vi "BNAL RADAR graph Formation.vi"(8 "Cutted Sample Sequence":string="TCTAGACTATCTCACTCTCAGATGAGATCGATAGATCAGT", 9 "Level Composition":string[](array[string]), 11 "Assigned#_CL":T1) -> (0 "Base_Tag_Array":string[](array[string]), 1 "Base_Com_Array":i32[](array[numeric]), 2 "Table Cluster":T2, 3 "Radar graph cluster":T3)   [LabVIEW 2018]
uses:
  a6b6b03c-adef-4b05-a669-847ce0550db9.vi
  4a9d2bae-dd06-40cf-8326-d887beb1304b.vi
  f1d95cbe-b5e7-4193-9626-4301581f2f47.vi
  <vilib>/Array/Sort 2D Array - Pop Stack.vi
  <vilib>/Array/Sort 2D Array - Push Stack.vi
panel:
  out "Tri_N_sort_#":string[](array[string])
  out "Tri_P_sort_#":string[](array[string])
  out "Di_N_sort_#":string[](array[string])
  out "Di_P_sort_#":string[](array[string])
  out "Mono_N_sort_#":string[](array[string])
  out "Mono_P_sort_#":string[](array[string])
  out "Tri Table":string[][](table)
  out "Di Table":string[][](table)
  out "Mono Table":string[][](table)
  out "Mono_N_sort_B":string[](array[string])
  out "Mono_P_sort_B":string[](array[string])
  out "Mono_P_sort_[%]":string[](array[string])
  out "Mono_N_sort_[%]":string[](array[string])
  out "Tri_N_sort_B":string[](array[string])
  out "Tri_P_sort_B":string[](array[string])
  out "Tri_P_sort_[%]":string[](array[string])
  out "Tri_N_sort_[%]":string[](array[string])
  out "Di_N_sort_B":string[](array[string])
  out "Di_P_sort_B":string[](array[string])
  out "Di_P_sort_[%]":string[](array[string])
  out "Di_N_sort_[%]":string[](array[string])
  out "Tri_sort_B":string[](array[string])
  out "Tri_sort":dbl[](array[numeric])
  out "Tri_Assig-Th":dbl[](array[numeric])
  out "TriBase_Array_Tag":string[](array[string])
  out "Di_sort_B":string[](array[string])
  out "Di_sort":dbl[](array[numeric])
  out "Mono_sort_B":string[](array[string])
  out "Mono_sort":dbl[](array[numeric])
  out "DiBase_Array_Tag":string[](array[string])
  out "MonoBase_Array_Tag":string[](array[string])
  out "Di_MxR-Th":dbl[](array[numeric])
  out "Mono_MxR-Th":dbl[](array[numeric])
  out "Di_Assig-Th":dbl[](array[numeric])
  out "Mono_Assig-Th":dbl[](array[numeric])
  out "Tri_Theory[%]":dbl[](array[numeric])
  out "Di_Theory[%]":dbl[](array[numeric])
  out "Mono_Theory[%]":dbl[](array[numeric])
  out "Tri_MxRight[%]":dbl[](array[numeric])
  out "Di_MxRight[%]":dbl[](array[numeric])
  out "Mono_MxRight[%]":dbl[](array[numeric])
  out "Tri_Assigned[%]":dbl[](array[numeric])
  out "Di_Assigned[%]":dbl[](array[numeric])
  out "Mono_Assigned[%]":dbl[](array[numeric])
  out "Tri_MxRight#":i32[](array[numeric])
  out "Di_MxRight#":i32[](array[numeric])
  out "Mono_MxRight#":i32[](array[numeric])
  out "Tri_Assigned#":i32[](array[numeric])
  out "Di_Assigned#":i32[](array[numeric])
  out "Mono_Assigned#":i32[](array[numeric])
  out "Radar Plot_XXX":picture
  out "Radar Plot_XX":picture
  out "Radar_X":picture
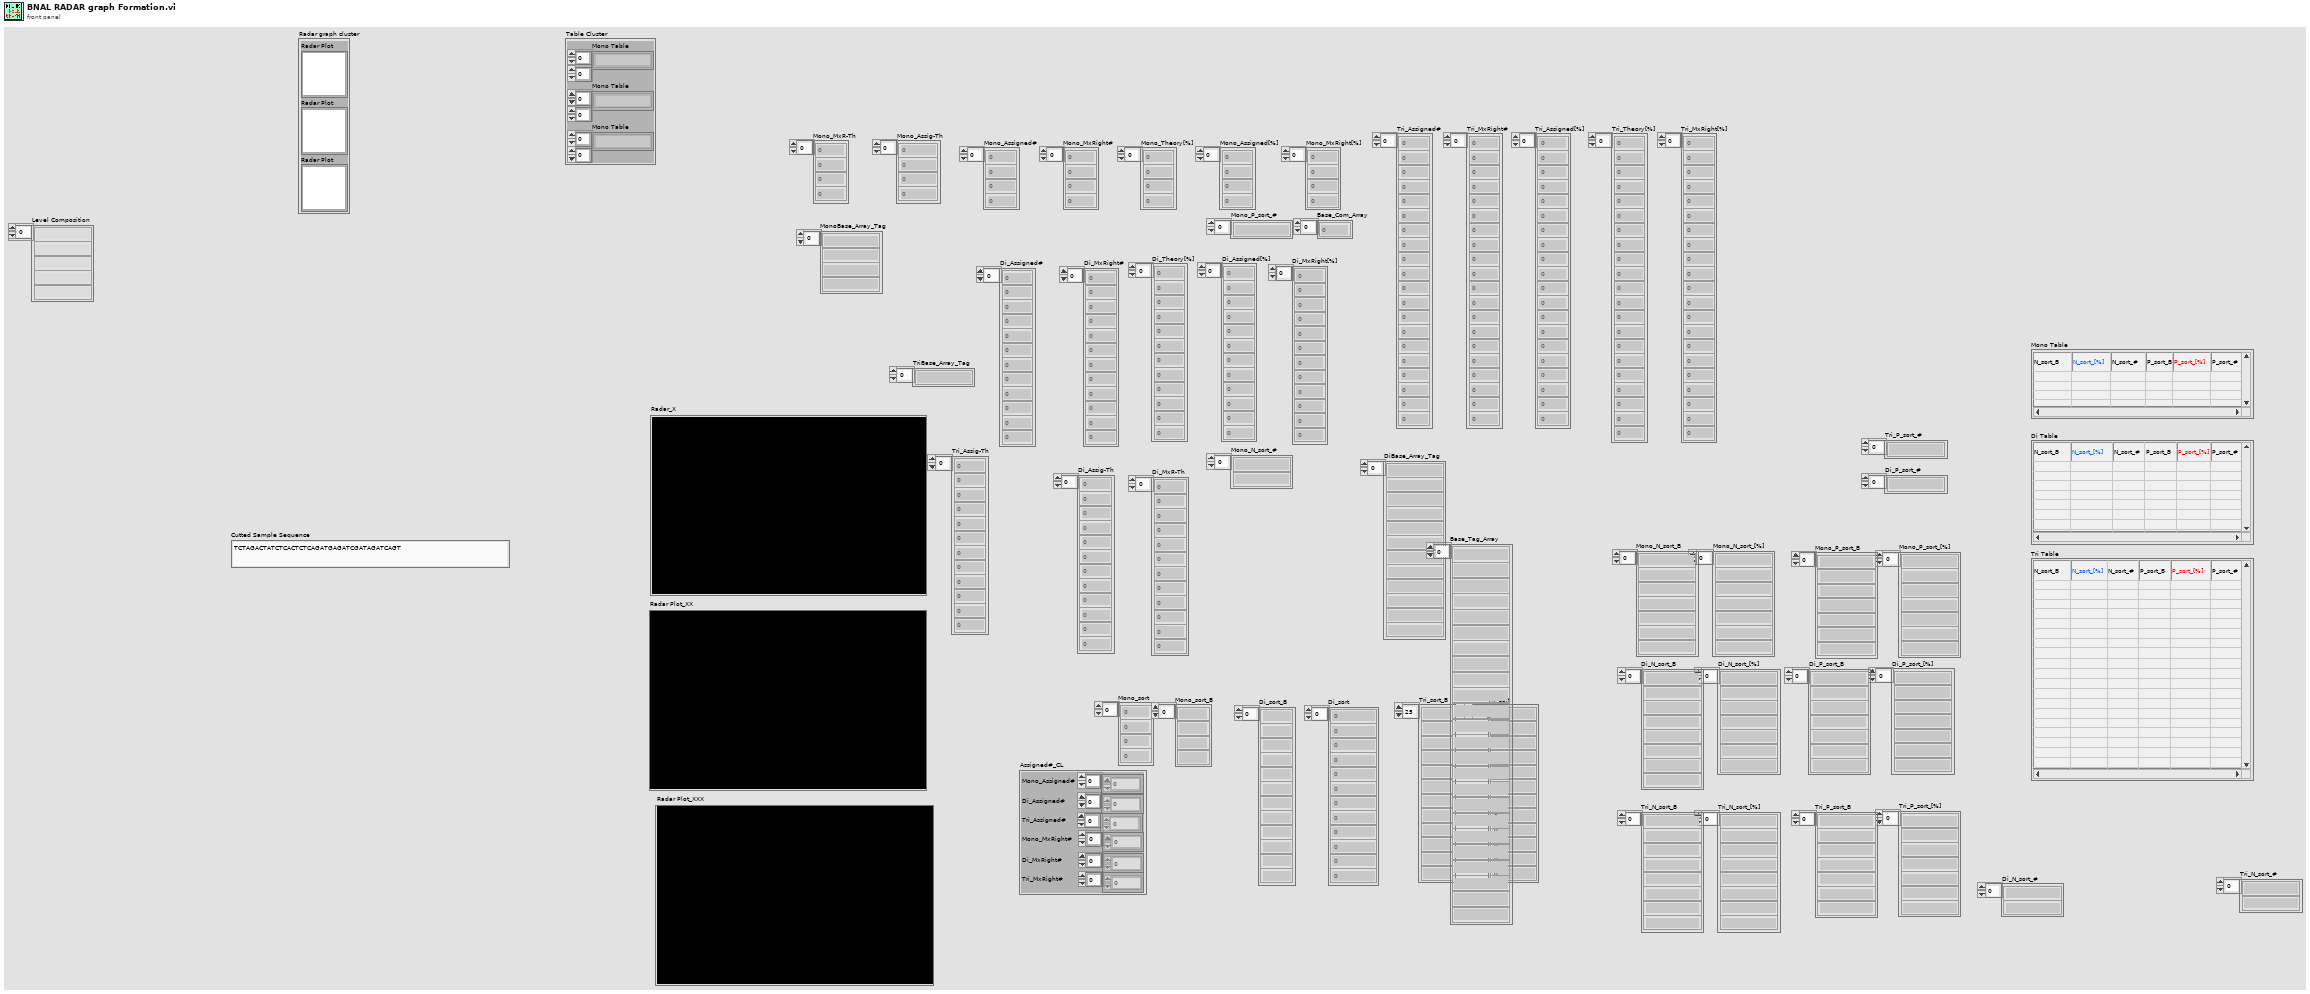
[diagram p1: front panel]
types:
  T1 = cluster{"Mono_Assigned#":i32[], "Di_Assigned#":i32[], "Tri_Assigned#":i32[], "Tri_MxRight#":i32[], "Di_MxRight#":i32[], "Mono_MxRight#":i32[]}
  T2 = cluster{"Mono Table":string[][], "Mono Table":string[][], "Mono Table":string[][]}
  T3 = cluster{"Radar Plot":picture, "Radar Plot":picture, "Radar Plot":picture}
  T4 = cluster{"MonoBase_Array_Tag":string[], "DiBase_Array_Tag":string[], "TriBase_Array_Tag":string[]}
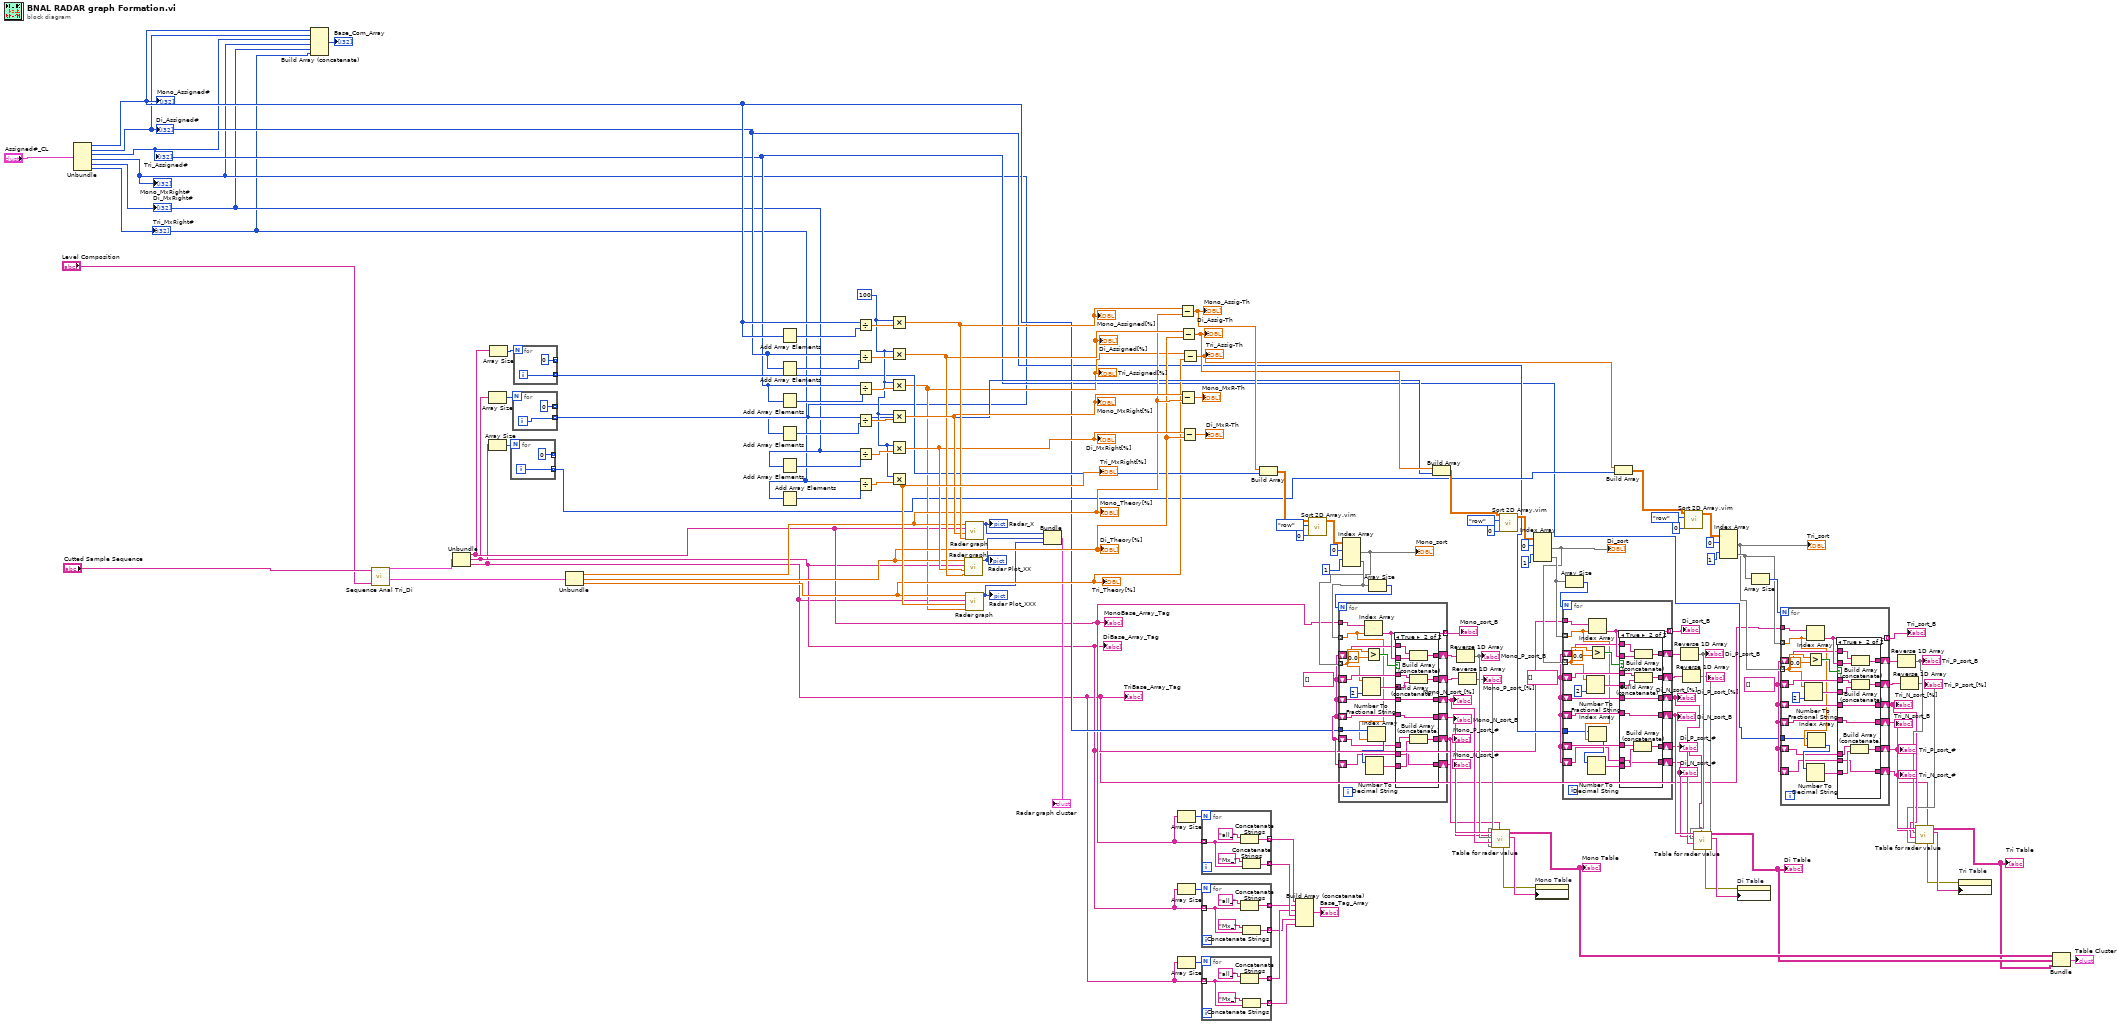
[diagram p0: block diagram]
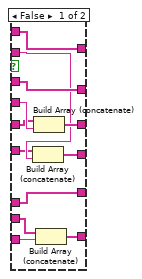
[diagram p2: hidden frame]
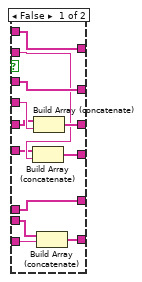
[diagram p3: hidden frame]
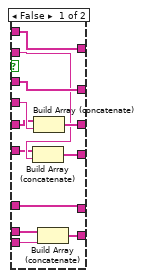
[diagram p4: hidden frame]
diagram:
  w38 = string[] []
  w36 = string[] []
  w37 = string[] []
  w110 = 100
  n1 = Unbundle("Assigned#_CL") -> ("Mono_Assigned#"=w20:i32[], "Di_Assigned#"=w19:i32[], "Tri_Assigned#"=w18:i32[], "Tri_MxRight#"=w17:i32[], "Di_MxRight#"=w16:i32[], "Mono_MxRight#"=w15:i32[])
  "Mono_Assigned#" <- w20
  "Di_Assigned#" <- w19
  "Tri_Assigned#" <- w18
  "Mono_MxRight#" <- w17
  "Di_MxRight#" <- w16
  "Tri_MxRight#" <- w15
  n2 = Build Array (concatenate)(w20, w19, w18, w17, w16, w15) -> (→"Base_Com_Array":i32[])
  n3 = call "Sequence Anal Tri_Di.vi"("Level Composition"="Level Composition", "String"="Cutted Sample Sequence") -> ("B%Number"=w127:cluster{dbl[], dbl[], dbl[]}, "Base Tag"=w128:T4)  [unwired: 7 in, 1 out]
  n4 = Unbundle(w128) -> ("MonoBase_Array_Tag"=w3:string[], "DiBase_Array_Tag"=w2:string[], "TriBase_Array_Tag"=w1:string[])
  "MonoBase_Array_Tag" <- w3
  "DiBase_Array_Tag" <- w2
  "TriBase_Array_Tag" <- w1
  n5 = Array Size(array=w2) -> (size(s)=w118:i32)
  n6 = Array Size(array=w1) -> (size(s)=w117:i32)
  n7 = Array Size(array=w3) -> (size(s)=w119:i32)
  n8 = for {
    N: w117 -> [_]
    tunnel: [0 ("index")] -> _ mode=indexing
    tunnel: [w130] -> w73 mode=indexing
    i -> [w130]
  }
  n9 = for {
    N: w118 -> [_]
    tunnel: [0 ("index")] -> _ mode=indexing
    tunnel: [w132] -> w91 mode=indexing
    i -> [w132]
  }
  n10 = for {
    N: w119 -> [_]
    tunnel: [0 ("index")] -> _ mode=indexing
    tunnel: [w134] -> w99 mode=indexing
    i -> [w134]
  }
  n11 = Unbundle(w127) -> (w102:dbl[], w101:dbl[], w81:dbl[])
  "Mono_Theory[%]" <- w102
  "Di_Theory[%]" <- w101
  "Tri_Theory[%]" <- w81
  n12 = Add Array Elements(numeric array=w20) -> (sum=w126:i32)
  n13 = Add Array Elements(numeric array=w19) -> (sum=w124:i32)
  n14 = Add Array Elements(numeric array=w18) -> (sum=w123:i32)
  n15 = Add Array Elements(numeric array=w17) -> (sum=w116:i32)
  n16 = Add Array Elements(numeric array=w16) -> (sum=w114:i32)
  n17 = Add Array Elements(numeric array=w15) -> (sum=w113:i32)
  n18 = Divide(x=w20, y=w126) -> (x/y=w125:dbl[])
  n19 = Divide(x=w19, y=w124) -> (x/y=w122:dbl[])
  n20 = Divide(x=w18, y=w123) -> (x/y=w121:dbl[])
  n21 = Divide(x=w17, y=w116) -> (x/y=w115:dbl[])
  n22 = Divide(x=w16, y=w114) -> (x/y=w112:dbl[])
  n23 = Divide(x=w15, y=w113) -> (x/y=w111:dbl[])
  n24 = Multiply(x=w110, y=w125) -> (x*y=w108:dbl[])
  "Mono_Assigned[%]" <- w108
  n25 = Multiply(x=w110, y=w122) -> (x*y=w106:dbl[])
  "Di_Assigned[%]" <- w106
  n26 = Multiply(x=w110, y=w121) -> (x*y=w80:dbl[])
  "Tri_Assigned[%]" <- w80
  n27 = Multiply(x=w110, y=w115) -> (x*y=w107:dbl[])
  "Mono_MxRight[%]" <- w107
  n28 = Multiply(x=w110, y=w112) -> (x*y=w104:dbl[])
  "Di_MxRight[%]" <- w104
  n29 = Multiply(x=w110, y=w111) -> (x*y=w109:dbl[])
  "Tri_MxRight[%]" <- w109
  n30 = call "Rader graph.vi"("Real B_Comp (NR)"=w106, "Real B_Comp (RR)"=w104, "XBase_Array_Tag"=w2, "Theory B_Comp"=w101) -> ("Radar Plot"=w28:picture)  [unwired: 7 in]
  "Radar Plot_XX" <- w28
  n31 = call "Rader graph.vi"("Real B_Comp (NR)"=w108, "Real B_Comp (RR)"=w107, "XBase_Array_Tag"=w3, "Theory B_Comp"=w102) -> ("Radar Plot"=w29:picture)  [unwired: 7 in]
  "Radar_X" <- w29
  n32 = call "Rader graph.vi"("Real B_Comp (NR)"=w80, "Real B_Comp (RR)"=w109, "XBase_Array_Tag"=w1, "Theory B_Comp"=w81) -> ("Radar Plot"=w27:picture)  [unwired: 7 in]
  "Radar Plot_XXX" <- w27
  n33 = Bundle("Radar Plot"=w29, "Radar Plot"=w28, "Radar Plot"=w27) -> (→"Radar graph cluster":T3)  [unwired: 1 in]
  n34 = Array Size(array=w3) -> (size(s)=w13:i32)
  n35 = Array Size(array=w2) -> (size(s)=w9:i32)
  n36 = Array Size(array=w1) -> (size(s)=w8:i32)
  n37 = Subtract(x=w108, y=w102) -> (x-y=w100:dbl[])
  "Mono_Assig-Th" <- w100
  n38 = Subtract(x=w107, y=w102) -> (x-y=→"Mono_MxR-Th":dbl[])
  n39 = Subtract(x=w106, y=w101) -> (x-y=w92:dbl[])
  "Di_Assig-Th" <- w92
  n40 = Subtract(x=w104, y=w101) -> (x-y=→"Di_MxR-Th":dbl[])
  n41 = Subtract(x=w80, y=w81) -> (x-y=w74:dbl[])
  "Tri_Assig-Th" <- w74
  n42 = for {
    N: w13 -> [_]
    tunnel: w3 -> [w136] mode=indexing
    tunnel: [w139] -> w12 mode=indexing
    tunnel: [w138] -> w10 mode=indexing
    n43 = Concatenate Strings("all_" ("string"), w136) -> (w139:string)
    n44 = Concatenate Strings("Mx_" ("string"), w136) -> (w138:string)
  }
  n45 = for {
    N: w9 -> [_]
    tunnel: w2 -> [w141] mode=indexing
    tunnel: [w144] -> w7 mode=indexing
    tunnel: [w143] -> w5 mode=indexing
    n46 = Concatenate Strings("all_" ("string"), w141) -> (w144:string)
    n47 = Concatenate Strings("Mx_" ("string"), w141) -> (w143:string)
  }
  n48 = for {
    N: w8 -> [_]
    tunnel: w1 -> [w146] mode=indexing
    tunnel: [w149] -> w6 mode=indexing
    tunnel: [w148] -> w4 mode=indexing
    n49 = Concatenate Strings("all_" ("string"), w146) -> (w149:string)
    n50 = Concatenate Strings("Mx_" ("string"), w146) -> (w148:string)
  }
  n51 = Build Array(w100, w99) -> (w98:dbl[][])
  n52 = Build Array (concatenate)(w12, w7, w6, w10, w5, w4) -> (→"Base_Tag_Array":string[])
  n53 = call "Sort 2D Array.vim"("index"=0, "dimension to index (column)"=enum16{"column", "row"}."row", "2D array"=w98) -> ("sorted 2D array"=w95:dbl[][])  [unwired: 7 in, 1 out]
  n54 = Index Array(array=w95, index (row) #1=0 ("index (row)"), index (row) #2=1 ("disabled index (col)")) -> (element #1=w57:dbl[], element #2=w58:dbl[])  [unwired: 2 in]
  "Mono_sort" <- w57
  n55 = Array Size(array=w58) -> (size(s)=w59:i32)
  n56 = for {
    N: w59 -> [_]
    tunnel: w3 -> [w173]
    tunnel: w58 -> [w157] mode=indexing
    tunnel: [w163] -> w60 mode=indexing
    shift-right: [w168] -> w62
    shift-left: w38 -> [w167]
    shift-right: [w166] -> w54
    shift-left: w38 -> [w165]
    tunnel: w57 -> [w164] mode=indexing
    shift-right: [w162] -> w61
    shift-left: w38 -> [w161]
    shift-right: [w160] -> w56
    shift-left: w38 -> [w159]
    tunnel: w20 -> [w158]
    shift-right: [w154] -> w35
    shift-left: w38 -> [w153]
    shift-right: [w152] -> w34
    shift-left: w38 -> [w151]
    n57 = Number To Fractional String(number=w164, precision (6)=i16 2) -> (F-format string=w169:string)  [unwired: 2 in]
    n58 = Index Array(array=w173, index=w157) -> (element=w163:string)
    n59 = Greater?(x=w164, y=0.0) -> (0:w172:bool)
    n60 = Index Array(array=w158, index=w157) -> (element=w156:i32)
    n61 = Number To Decimal String(number=w156) -> (decimal integer string=w155:string)  [unwired: 1 in]
    n62 = case shown="True" w172 {
      tunnel: w169 -> [w184 w197]
      tunnel: [w185 w196] -> w168
      tunnel: w167 -> [w185 w195]
      tunnel: [w183 w194] -> w166
      tunnel: w165 -> [w182 w194]
      tunnel: w163 -> [w180 w193]
      tunnel: [w181 w192] -> w162
      tunnel: w161 -> [w181 w191]
      tunnel: [w179 w190] -> w160
      tunnel: w159 -> [w178 w190]
      tunnel: w155 -> [w176 w189]
      tunnel: [w177 w188] -> w154
      tunnel: w153 -> [w177 w187]
      tunnel: [w175 w186] -> w152
      tunnel: w151 -> [w174 w186]
      frame False {
        n63 = Build Array (concatenate)(w178, w180) -> (w179:string[])
        n64 = Build Array (concatenate)(w182, w184) -> (w183:string[])
        n65 = Build Array (concatenate)(w174, w176) -> (w175:string[])
      }
      frame True {
        n66 = Build Array (concatenate)(w187, w189) -> (w188:string[])
        n67 = Build Array (concatenate)(w191, w193) -> (w192:string[])
        n68 = Build Array (concatenate)(w195, w197) -> (w196:string[])
      }
    }
  }
  "Mono_sort_B" <- w60
  "Mono_N_sort_[%]" <- w54
  "Mono_N_sort_B" <- w56
  "Mono_P_sort_#" <- w35
  "Mono_N_sort_#" <- w34
  n69 = Build Array(w92, w91) -> (w82:dbl[][])
  n70 = Reverse 1D Array(array=w61) -> (reversed array=w55:string[])
  "Mono_P_sort_B" <- w55
  n71 = Reverse 1D Array(array=w62) -> (reversed array=w53:string[])
  "Mono_P_sort_[%]" <- w53
  n72 = call "Table for rader value.vi"("N_sort_#"=w34, "P_sort_#"=w35, "P_sort_[%]"=w53, "N_sort_[%]"=w54, "P_sort_B"=w55, "N_sort_B"=w56) -> ("Mono Table Tag"=w52:string[], "Mono Table"=w25:string[][], "error out"=w51:errorcluster)  [unwired: 3 in]
  "Mono Table" <- w25
  n73 = call "Sort 2D Array.vim"("index"=0, "dimension to index (column)"=enum16{"column", "row"}."row", "2D array"=w82) -> ("sorted 2D array"=w88:dbl[][])  [unwired: 7 in, 1 out]
  n74 = Index Array(array=w88, index (row) #1=0 ("index (row)"), index (row) #2=1 ("disabled index (col)")) -> (element #1=w71:dbl[], element #2=w85:dbl[])  [unwired: 2 in]
  "Di_sort" <- w71
  n75 = property on="Mono Table" class="Tbl (strict)"(error in=w51, "Column Headers[]"=w52) -> ()  [unwired: 1 in, 2 out]
  n76 = Array Size(array=w85) -> (size(s)=w84:i32)
  n77 = for {
    N: w84 -> [_]
    tunnel: w2 -> [w220]
    tunnel: w85 -> [w205] mode=indexing
    tunnel: [w210] -> w83 mode=indexing
    shift-right: [w215] -> w70
    shift-left: w37 -> [w214]
    shift-right: [w213] -> w46
    shift-left: w37 -> [w212]
    tunnel: w71 -> [w211] mode=indexing
    shift-right: [w209] -> w69
    shift-left: w37 -> [w208]
    shift-right: [w207] -> w48
    shift-left: w37 -> [w206]
    tunnel: w19 -> [w204]
    shift-right: [w200] -> w33
    shift-left: w37 -> [w203]
    shift-right: [w199] -> w32
    shift-left: w37 -> [w198]
    n78 = Number To Fractional String(number=w211, precision (6)=i16 2) -> (F-format string=w216:string)  [unwired: 2 in]
    n79 = Index Array(array=w220, index=w205) -> (element=w210:string)
    n80 = Index Array(array=w204, index=w205) -> (element=w202:i32)
    n81 = Number To Decimal String(number=w202) -> (decimal integer string=w201:string)  [unwired: 1 in]
    n82 = Greater?(x=w211, y=0.0) -> (0:w219:bool)
    n83 = case shown="True" w219 {
      tunnel: w216 -> [w231 w244]
      tunnel: [w232 w243] -> w215
      tunnel: w214 -> [w232 w242]
      tunnel: [w230 w241] -> w213
      tunnel: w212 -> [w229 w241]
      tunnel: w210 -> [w227 w240]
      tunnel: [w228 w239] -> w209
      tunnel: w208 -> [w228 w238]
      tunnel: [w226 w237] -> w207
      tunnel: w206 -> [w225 w237]
      tunnel: w203 -> [w224 w236]
      tunnel: w201 -> [w223 w235]
      tunnel: [w224 w234] -> w200
      tunnel: [w222 w233] -> w199
      tunnel: w198 -> [w221 w233]
      frame False {
        n84 = Build Array (concatenate)(w225, w227) -> (w226:string[])
        n85 = Build Array (concatenate)(w229, w231) -> (w230:string[])
        n86 = Build Array (concatenate)(w221, w223) -> (w222:string[])
      }
      frame True {
        n87 = Build Array (concatenate)(w236, w235) -> (w234:string[])
        n88 = Build Array (concatenate)(w238, w240) -> (w239:string[])
        n89 = Build Array (concatenate)(w242, w244) -> (w243:string[])
      }
    }
  }
  "Di_sort_B" <- w83
  "Di_N_sort_[%]" <- w46
  "Di_N_sort_B" <- w48
  "Di_P_sort_#" <- w33
  "Di_N_sort_#" <- w32
  n90 = Build Array(w74, w73) -> (w72:dbl[][])
  n91 = Reverse 1D Array(array=w69) -> (reversed array=w47:string[])
  "Di_P_sort_B" <- w47
  n92 = Reverse 1D Array(array=w70) -> (reversed array=w45:string[])
  "Di_P_sort_[%]" <- w45
  n93 = call "Sort 2D Array.vim"("index"=0, "dimension to index (column)"=enum16{"column", "row"}."row", "2D array"=w72) -> ("sorted 2D array"=w77:dbl[][])  [unwired: 7 in, 1 out]
  n94 = call "Table for rader value.vi"("N_sort_#"=w32, "P_sort_#"=w33, "P_sort_[%]"=w45, "N_sort_[%]"=w46, "P_sort_B"=w47, "N_sort_B"=w48) -> ("Mono Table Tag"=w50:string[], "Mono Table"=w24:string[][], "error out"=w49:errorcluster)  [unwired: 3 in]
  "Di Table" <- w24
  n95 = Index Array(array=w77, index (row) #1=0 ("index (row)"), index (row) #2=1 ("disabled index (col)")) -> (element #1=w64:dbl[], element #2=w65:dbl[])  [unwired: 2 in]
  "Tri_sort" <- w64
  n96 = property on="Di Table" class="Tbl (strict)"(error in=w49, "Column Headers[]"=w50) -> ()  [unwired: 1 in, 2 out]
  n97 = Array Size(array=w65) -> (size(s)=w66:i32)
  n98 = for {
    N: w66 -> [_]
    tunnel: w1 -> [w267]
    tunnel: w65 -> [w252] mode=indexing
    tunnel: [w257] -> w63 mode=indexing
    shift-right: [w262] -> w68
    shift-left: w36 -> [w261]
    shift-right: [w260] -> w40
    shift-left: w36 -> [w259]
    tunnel: w64 -> [w258] mode=indexing
    shift-right: [w256] -> w67
    shift-left: w36 -> [w255]
    shift-right: [w254] -> w42
    shift-left: w36 -> [w253]
    tunnel: w18 -> [w251]
    shift-right: [w248] -> w31
    shift-left: w36 -> [w247]
    shift-right: [w246] -> w30
    shift-left: w36 -> [w245]
    n99 = Number To Fractional String(number=w258, precision (6)=i16 2) -> (F-format string=w263:string)  [unwired: 2 in]
    n100 = Index Array(array=w267, index=w252) -> (element=w257:string)
    n101 = Greater?(x=w258, y=0.0) -> (0:w266:bool)
    n102 = Index Array(array=w251, index=w252) -> (element=w250:i32)
    n103 = Number To Decimal String(number=w250) -> (decimal integer string=w249:string)  [unwired: 1 in]
    n104 = case shown="True" w266 {
      tunnel: w263 -> [w278 w291]
      tunnel: [w279 w290] -> w262
      tunnel: w261 -> [w279 w289]
      tunnel: [w277 w288] -> w260
      tunnel: w259 -> [w276 w288]
      tunnel: w257 -> [w274 w287]
      tunnel: [w275 w286] -> w256
      tunnel: w255 -> [w275 w285]
      tunnel: [w273 w284] -> w254
      tunnel: w253 -> [w272 w284]
      tunnel: w249 -> [w270 w283]
      tunnel: [w271 w282] -> w248
      tunnel: w247 -> [w271 w281]
      tunnel: [w269 w280] -> w246
      tunnel: w245 -> [w268 w280]
      frame False {
        n105 = Build Array (concatenate)(w272, w274) -> (w273:string[])
        n106 = Build Array (concatenate)(w276, w278) -> (w277:string[])
        n107 = Build Array (concatenate)(w268, w270) -> (w269:string[])
      }
      frame True {
        n108 = Build Array (concatenate)(w281, w283) -> (w282:string[])
        n109 = Build Array (concatenate)(w285, w287) -> (w286:string[])
        n110 = Build Array (concatenate)(w289, w291) -> (w290:string[])
      }
    }
  }
  "Tri_sort_B" <- w63
  "Tri_N_sort_[%]" <- w40
  "Tri_N_sort_B" <- w42
  "Tri_P_sort_#" <- w31
  "Tri_N_sort_#" <- w30
  n111 = Reverse 1D Array(array=w67) -> (reversed array=w41:string[])
  "Tri_P_sort_B" <- w41
  n112 = Reverse 1D Array(array=w68) -> (reversed array=w39:string[])
  "Tri_P_sort_[%]" <- w39
  n113 = call "Table for rader value.vi"("N_sort_#"=w30, "P_sort_#"=w31, "P_sort_[%]"=w39, "N_sort_[%]"=w40, "P_sort_B"=w41, "N_sort_B"=w42) -> ("Mono Table Tag"=w44:string[], "Mono Table"=w23:string[][], "error out"=w43:errorcluster)  [unwired: 3 in]
  "Tri Table" <- w23
  n114 = property on="Tri Table" class="Tbl (strict)"(error in=w43, "Column Headers[]"=w44) -> ()  [unwired: 1 in, 2 out]
  n115 = Bundle("Mono Table"=w25, "Mono Table"=w24, "Mono Table"=w23) -> (→"Table Cluster":T2)  [unwired: 1 in]
